vi "Message over the network.vi"(0 "Guardian in":refnum<class "Guardian.lvclass">, 1 "Destination GD ID":string, 2 "Target ID (uService ID or \"Guardian\")":string, 3 "Message":string, 4 "Data":variant, 5 "error in (no error)":errorcluster) -> (14 "Guardian out":refnum<class "Guardian.lvclass">, 19 "error out":errorcluster)   [LabVIEW 2020, in "TALOS.lvlib" / "Guardian.lvlib" / "Guardian.lvclass"]
doc: "To send a message to a Guardian, type \"Guardian\" into the Target ID field."
uses:
  Guardian.lvclass
  Guardian.lvclass/Guardian.ctl
  Internal uServices/System uServices/TCP Writer/TCP Writer/TCP Message Internal Composition.ctl
  Ancestor/Ancestor/Ancestor.lvclass/Ancestor.ctl
  Support VIs/Generate Error.vi
  FGV/Error Memory/Get Error Description.vi
  Support VIs/Get PC name.vi
  Ancestor/Ancestor/Read ID.vi
  Support VIs/Get Class Name.vi
  <vilib>/Utility/error.llb/Clear Errors.vi
  FGV/Error Memory/Error Memory Core.vi
  <vilib>/AdvancedString/Delimited String to 1D String Array.vi
  Support VIs/Circus Root Path.vi
  FGV/Error Memory/Error Crt Lvl checker.vi
  FGV/Error Memory/Error Memory Core.vi/40c8088d-b597-4017-91af-faa98e00292e.vi
  FGV/Error Memory/Error Memory Core.vi/d4a3ab98-063c-4e44-b43d-fbdcfe6c2be2.vi
  Support VIs/Global Memory.vi
  <vilib>/Utility/LVClass/Get LV Class Name.vi
  Support VIs/Is in Packed Library.vi
  Support VIs/TALOS Root path.vi
  Support VIs/Read CSV worksheet.vi
  <vilib>/Utility/error.llb/General Error Handler.vi
  Support VIs/Error Log.vi
  Ancestor/Ancestor/Ancestor.lvclass
  <vilib>/Comparison/Equal/Equal Functor/Equal Functor.lvclass
  Classes/Guardian List/Guardian List.lvclass
  Internal uServices/System uServices/TCP Writer/TCP Writer/TCP Writer.lvclass
  TALOS.lvlib
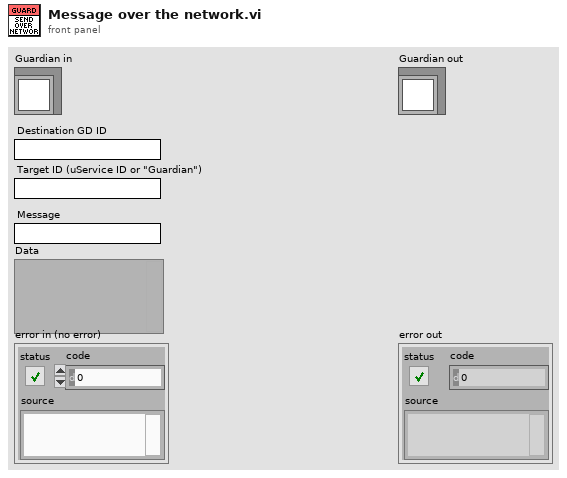
[diagram p1: front panel]
types:
  T1 = typedef "TALOS.lvlib/TCP Writer.lvlib/TCP Writer.lvclass/TCP Message Internal Composition.ctl" = cluster{"uS/GD ID":string, "Message":string, "Data":variant}
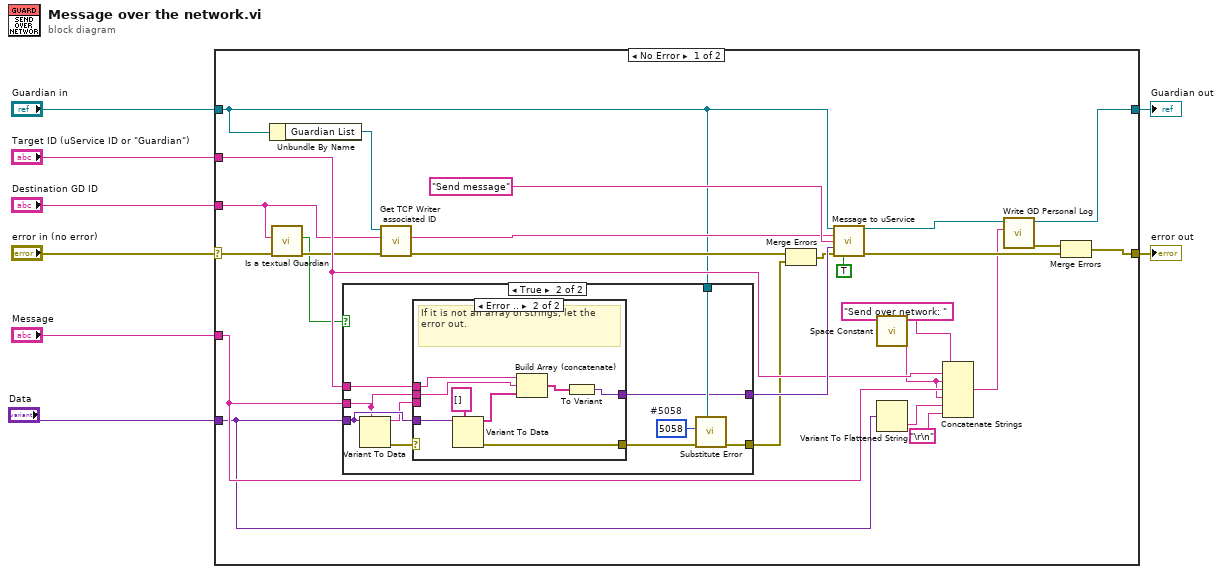
[diagram p0: block diagram]
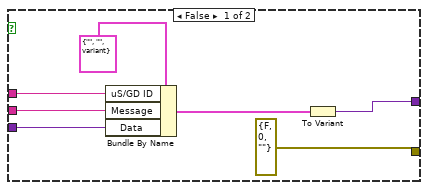
[diagram p2: hidden frame]
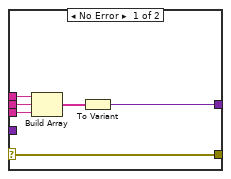
[diagram p3: hidden frame]
diagram:
  n1 = case shown="No Error" "error in (no error)" {
    selector: "error in (no error)" -> [w15 w67]
    tunnel: [w25 w67] -> w8
    tunnel: "Guardian in" -> [w11 w66]
    tunnel: "Data" -> [w20 _]
    tunnel: "Message" -> [w21 _]
    tunnel: "Target ID (uService ID or \"Guardian\")" -> [w22 _]
    tunnel: "Destination GD ID" -> [w14 _]
    tunnel: [w27 w66] -> w1
    frame No Error {
      n2 = Unbundle By Name(w11) -> ("Guardian List"=w29:refnum<class "Guardian List.lvclass">)
      n3 = call "Is a textual Guardian.vi"("error in (no error)"=w15, "Target GD ID"=w14) -> ("error out"=w13:errorcluster, "Textual?"=w12:bool)  [unwired: 8 in]
      n4 = case shown="True" w12 {
        tunnel: [w36 w45] -> w33
        tunnel: w22 -> [w39 w47]
        tunnel: w21 -> [w38 w46]
        tunnel: w20 -> [w37 w51]
        tunnel: w11 -> [_ w49]
        tunnel: [errorcluster {"status"=FALSE, "code"=0, "source"=""} ("error out") w48] -> w9
        frame False {
          n5 = Bundle By Name(cluster=T1 {"uS/GD ID"="", "Message"="", "Data"=variant}, "uS/GD ID"=w39, "Message"=w38, "Data"=w37) -> (w41:T1)
          n6 = To Variant(anything=w41) -> (Variant=w36:variant)
        }
        frame True {
          w50 = 5058  # #5058
          n7 = Variant To Data(type=w46, Variant=w51) -> (data=w44:string, error out=w43:errorcluster)  [unwired: 1 in]
          n8 = case shown="Error .." w43 {
            selector: w43 -> [w52 _]
            tunnel: w47 -> [w57 w62]
            tunnel: w46 -> [w56 w61]
            tunnel: [w54 w58] -> w45
            tunnel: w44 -> [w53 _]
            tunnel: [w52 w63] -> w42
            tunnel: w51 -> [_ w65]
            frame No Error {
              n9 = Build Array(w57, w56, w53) -> (w55:string[])
              n10 = To Variant(anything=w55) -> (Variant=w54:variant)
            }
            frame Error {
              # "If it is not an array of strings, let the error out."
              n11 = Variant To Data(type=string[] [], Variant=w65) -> (data=w60:string[], error out=w63:errorcluster)  [unwired: 1 in]
              n12 = Build Array (concatenate)(w62, w61, w60) -> (w59:string[])
              n13 = To Variant(anything=w59) -> (Variant=w58:variant)
            }
          }
          n14 = call "Substitute Error.vi"("LabVIEW Object"=w49, "error in (no error)"=w42, "Error Code"=w50) -> ("error out"=w48:errorcluster)  [unwired: 8 in]
        }
      }
      n15 = call-dynamic "Get TCP Writer associated ID.vi"("error in (no error)"=w13, "ID"=w14, "Guardian List in"=w29) -> ("error out"=w30:errorcluster, "TCP Writer associated ID"=w31:string)  [unwired: 6 in, 1 out]
      n16 = Merge Errors(w30, w9) -> (w10:errorcluster)
      n17 = call "Message to uService.vi"("Guardian in"=w11, "uService ID"=w31, "Message"="Send message" ("Item Name"), "Data"=w33, "error in (no error)"=w10, "Locale?"=TRUE) -> ("Guardian out"=w28:refnum<class "Guardian.lvclass">, "error out"=w24:errorcluster)  [unwired: 8 in]
      n18 = call <vilib>:"Space Constant.vi"() -> ("String"=w17:string)
      n19 = Variant To Flattened String(Variant=w20) -> (data string=w19:string)  [unwired: 1 out]
      n20 = Concatenate Strings("Send over network: " ("string"), w22, w17, w21, w17, w19, "\r\n") -> (w18:string)
      n21 = call "Write GD Personal Log.vi"("String"=w18, "Guardian in"=w28) -> ("error out"=w26:errorcluster, "Guardian out"=w27:refnum<class "Guardian.lvclass">)  [unwired: 8 in]
      n22 = Merge Errors(w26, w24) -> (w25:errorcluster)
    }
    frame Error {
    }
  }
  "error out" <- w8
  "Guardian out" <- w1
